vi "PathPlanner_Path_Test.vi"(8 "error in (no error)":errorcluster) -> (0 "error out":errorcluster, 3 "All Passed":bool)   [LabVIEW 2019]
uses:
  <vilib>/Rock Robotics/WPI/ThirdParty/JAS_Junk/TrajLib/Rotation2d_CreateAngle.vi
  <vilib>/Rock Robotics/WPI/ThirdParty/MJansen/PathPlanner/VI/PathPlanner_Waypoint_AutoCtrlPoints.vi
  <vilib>/Rock Robotics/WPI/ThirdParty/JAS_Junk/TrajLib/Pose2d_getTranslation.vi
  <vilib>/Rock Robotics/WPI/ThirdParty/JAS_Junk/TrajLib/Pose2d_getRotation.vi
  <vilib>/Rock Robotics/WPI/ThirdParty/JAS_Junk/TrajLib/Conv_Deg_Radians.vi
  <vilib>/Rock Robotics/WPI/ThirdParty/JAS_Junk/TrajLib/Pose2d_New_TRRO.vi
  <vilib>/Rock Robotics/WPI/ThirdParty/MJansen/PathPlanner/VI/PathPlanner_Path_GetPoint.vi
  <vilib>/Rock Robotics/WPI/ThirdParty/MJansen/PathPlanner/VI/PathPlanner_PathPoint_GetAll.vi
  <vilib>/Rock Robotics/WPI/ThirdParty/MJansen/PathPlanner/VI/PathPlanner_Path_GetIdealStartingState.vi
  <vilib>/Rock Robotics/WPI/ThirdParty/MJansen/PathPlanner/VI/PathPlanner_IdealStartingState_GetAll.vi
  <vilib>/Rock Robotics/WPI/ThirdParty/MJansen/PathPlanner/VI/PathPlanner_Path_IsReversed.vi
  <vilib>/Rock Robotics/WPI/ThirdParty/JAS_Junk/TrajLib/Rotation2d_GetDegrees.vi
  <vilib>/Rock Robotics/WPI/ThirdParty/JAS_Junk/TrajLib/MathUtil_InputModulus.vi
  <vilib>/Rock Robotics/WPI/ThirdParty/MJansen/PathPlanner/VI/PathPlanner_Path_GetInitialHeading.vi
  <vilib>/Rock Robotics/WPI/ThirdParty/JAS_Junk/TrajLib/Translation2d_Minus.vi
  <vilib>/Rock Robotics/WPI/ThirdParty/JAS_Junk/TrajLib/Translation2d_Create_DistAng.vi
  <vilib>/Rock Robotics/WPI/ThirdParty/JAS_Junk/TrajLib/Translation2d_GetDistance.vi
  <vilib>/Rock Robotics/WPI/ThirdParty/MJansen/PathPlanner/VI/PathPlanner_Waypoint_AutoCtrlDistFactor.vi
  <vilib>/Rock Robotics/WPI/ThirdParty/JAS_Junk/TrajLib/Translation2d_Plus.vi
  <vilib>/Rock Robotics/WPI/ThirdParty/JAS_Junk/TrajLib/Rotation2d_GetRadians.vi
  <vilib>/Rock Robotics/WPI/ThirdParty/JAS_Junk/TrajLib/Translation2d_GetAngle.vi
  <vilib>/Rock Robotics/WPI/ThirdParty/JAS_Junk/TrajLib/Rotation2d_GetAngleCosSin.vi
  <vilib>/Rock Robotics/WPI/ThirdParty/JAS_Junk/TrajLib/Util_CalcDist.vi
  <vilib>/Rock Robotics/WPI/ThirdParty/JAS_Junk/TrajLib/Translation2d_GetXY.vi
  <vilib>/Rock Robotics/WPI/ThirdParty/JAS_Junk/TrajLib/Rotation2d_CreateXY.vi
  <vilib>/Rock Robotics/WPI/ThirdParty/JAS_Junk/TrajLib/Trajectory_Library.lvlib
  <vilib>/Rock Robotics/WPI/ThirdParty/MJansen/PathPlanner/PathPlanner24.lvlib
panel:
  out "Error 2":bool
  out "Error":bool
  out "Passed 3":bool
  out "Passed 2":bool
  out "Passed 1":bool
  # "DifferentialStartingPose"
  # "HolomonicStartingPoseSet"
  # "HolomonicStartingPose Null"
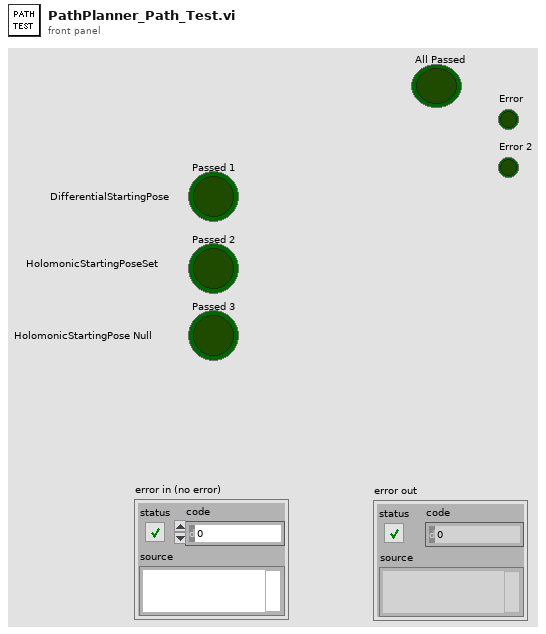
[diagram p1: front panel]
types:
  T1 = typedef "Trajectory_Library.lvlib/TRANSLATION2D.ctl" = cluster{"X":dbl, "Y":dbl}
  T2 = typedef "Trajectory_Library.lvlib/ROTATION2D.ctl" = cluster{"VALUE":dbl, "COS":dbl, "SIN":dbl}
  T3 = typedef "Trajectory_Library.lvlib/POSE2D.ctl" = cluster{"TRANSLATION":T1, "ROTATION":T2}
  T4 = typedef "PathPlanner24.lvlib/PathPlannerPathConstraints.ctl" = cluster{"MaxVelocityMps;":dbl, "MaxAccelerationMpsSq;":dbl, "MaxAngularVelRadPsEc;":dbl, "MaxAngularAccRadPSecSq":dbl, "Exists":bool, "Unlimited":bool, "NominalVoltageVolts":dbl}
  T5 = typedef "PathPlanner24.lvlib/PathPlannerGoalEndState.ctl" = cluster{"VelocityMPS":dbl, "Rotation":T2}
  T6 = typedef "PathPlanner24.lvlib/PathPlannerIdealStartingState.ctl" = cluster{"VelocityMPS":dbl, "Rotation":T2}
  T7 = typedef "PathPlanner24.lvlib/PathPlannerWaypoint.ctl" = cluster{"prevControl":T1, "anchor":T1, "nextControl":T1, "PrevExists":bool, "NextExists":bool}
  T8 = typedef "PathPlanner24.lvlib/PathPlannerPath.ctl" = cluster{"Reversed":bool, "RotationTargets":T9[], "ConstraintZones":T10[], "EventMarkers":T11[], "GlobalConstraints":T4, "GoalEndState":T5, "AllPoints":T14[], "Name":string, "Waypoints":T7[], "PointTowardsZones":T15[], "IdealStartingState":T6, "IsChoreoPath":bool, "PreventFlipping":bool}
  T9 = typedef "PathPlanner24.lvlib/PathPlannerRotationTarget.ctl" = cluster{"position":dbl, "rotation":T2, "Exists":bool}
  T10 = typedef "PathPlanner24.lvlib/PathPlannerConstraintsZone.ctl" = cluster{"minPosition":dbl, "maxPosition":dbl, "Constraints":T4, "Present":bool}
  T11 = typedef "PathPlanner24.lvlib/PathPlannerEventMarker.ctl" = cluster{"Position":dbl, "Command":T12, "TriggerName":string, "EndPosition":dbl}
  T12 = typedef "PathPlanner24.lvlib/PathPlannerCommandUtil.ctl" = cluster{"waitTime":dbl, "name":string, "pathName":string, "commands":cluster{"type":T13, "waitTime":dbl, "name":string, "pathName":string}[], "type":T13}
  T13 = typedef "PathPlanner24.lvlib/PathPlanner_CommandUtilType_ENUM.ctl" = enum16{"Unknown", "Wait", "Named", "Path", "Sequential", "Parallel", "Race", "Deadline"}
  T14 = typedef "PathPlanner24.lvlib/PathPlannerPathPoint.ctl" = cluster{"Position":T1, "DistAlongPath":dbl, "MaxV":dbl, "Constraints":T4, "RotationTarget":T9, "WaypointRelativePos":dbl}
  T15 = typedef "PathPlanner24.lvlib/PathPlannerPointTowardsZone.ctl" = cluster{"RotationOffset":T2, "Name":string, "TargetPosition":T1, "MinPosition":dbl, "MaxPosition":dbl}
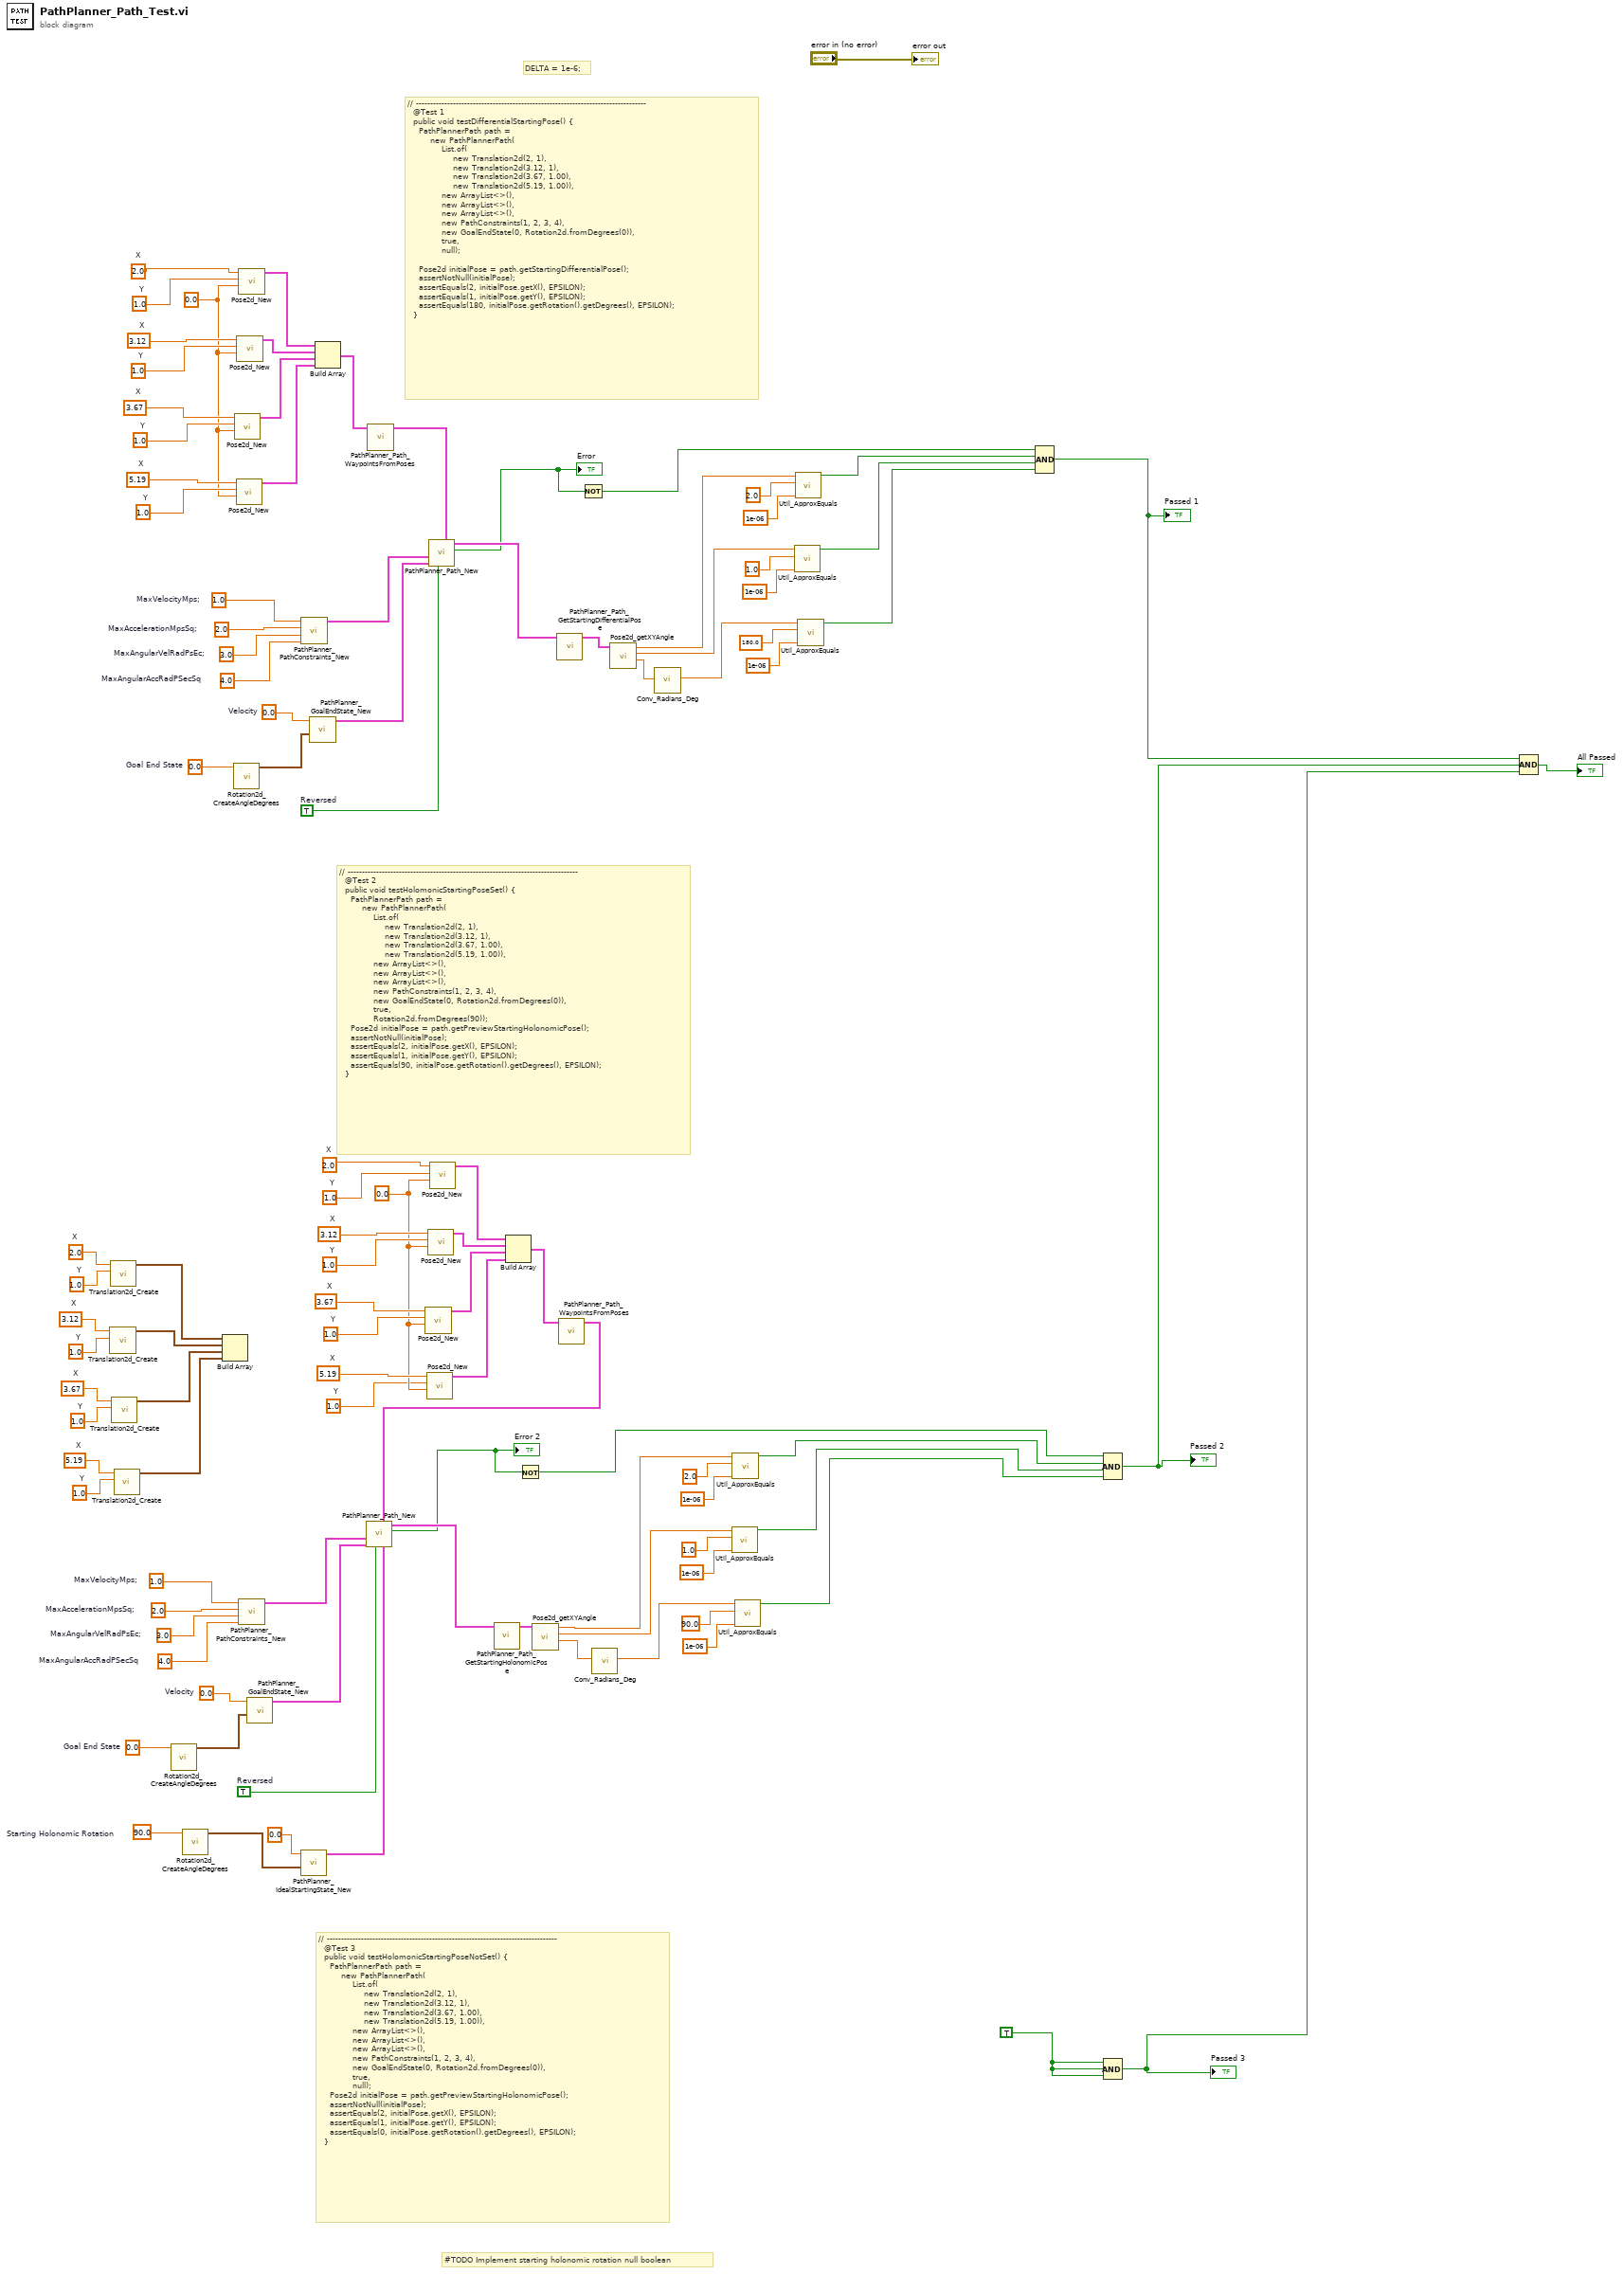
[diagram p0: block diagram]
diagram:
  w12 = 0.0 ("Heading")
  w13 = 5.19  # X
  w6 = 1.0  # Y
  w19 = 2.0  # X
  w18 = 1.0  # Y
  w15 = 3.67  # X
  w14 = 1.0  # Y
  w17 = 3.12  # X
  w16 = 1.0  # Y
  w27 = 0.0 ("Heading")
  w36 = TRUE
  w46 = 90.0  # Starting Holonomic Rotation
  w51 = 0.0  # Velocity
  w53 = 0.0  # Goal End State
  w54 = TRUE  # Reversed
  w60 = 5.19  # X
  w59 = 1.0  # Y
  w62 = 2.0  # X
  w61 = 1.0  # Y
  w64 = 3.67  # X
  w63 = 1.0  # Y
  w66 = 3.12  # X
  w65 = 1.0  # Y
  w72 = 1.0  # MaxVelocityMps;
  w73 = 2.0  # MaxAccelerationMpsSq;
  w74 = 3.0  # MaxAngularVelRadPsEc;
  w75 = 4.0  # MaxAngularAccRadPSecSq
  w87 = 0.0  # Velocity
  w89 = 0.0  # Goal End State
  w90 = TRUE  # Reversed
  w29 = 5.19  # X
  w28 = 1.0  # Y
  w35 = 2.0  # X
  w34 = 1.0  # Y
  w31 = 3.67  # X
  w30 = 1.0  # Y
  w33 = 3.12  # X
  w32 = 1.0  # Y
  w97 = 1.0  # MaxVelocityMps;
  w98 = 2.0  # MaxAccelerationMpsSq;
  w99 = 3.0  # MaxAngularVelRadPsEc;
  w100 = 4.0  # MaxAngularAccRadPSecSq
  # "#TODO Implement starting holonomic rotation null boolean"
  # "// ---------------------------------------------------------------------------------\n  @Test 3\n  public void testHolomonicStartingPoseNotSet() {\n    PathPlannerPath path =\n        new PathPlannerPath(\n            List.of(\n                new Translation2d(2, 1),\n                new Translation2d(3.12, 1),\n                new Translation2d(3.67, 1.00),\n                new Translation2d(5.19, 1.00)),\n            new ArrayList<>(),\n            new ArrayList<>(),\n            new ArrayList<>(),\n            new PathConstraints(1, 2, 3, 4),\n            new GoalEndState(0, Rotation2d.fromDegrees(0)),\n            true,\n            null);\n    Pose2d initialPose = path.getPreviewStartingHolonomicPose();\n    assertNotNull(initialPose);\n    assertEquals(2, initialPose.getX(), EPSILON);\n    assertEquals(1, initialPose.getY(), EPSILON);\n    assertEquals(0, initialPose.getRotation().getDegrees(), EPSILON);\n  }"
  # "// ---------------------------------------------------------------------------------\n  @Test 2\n  public void testHolomonicStartingPoseSet() {\n    PathPlannerPath path =\n        new PathPlannerPath(\n            List.of(\n                new Translation2d(2, 1),\n                new Translation2d(3.12, 1),\n                new Translation2d(3.67, 1.00),\n                new Translation2d(5.19, 1.00)),\n            new ArrayList<>(),\n            new ArrayList<>(),\n            new ArrayList<>(),\n            new PathConstraints(1, 2, 3, 4),\n            new GoalEndState(0, Rotation2d.fromDegrees(0)),\n            true,\n            Rotation2d.fromDegrees(90));\n    Pose2d initialPose = path.getPreviewStartingHolonomicPose();\n    assertNotNull(initialPose);\n    assertEquals(2, initialPose.getX(), EPSILON);\n    assertEquals(1, initialPose.getY(), EPSILON);\n    assertEquals(90, initialPose.getRotation().getDegrees(), EPSILON);\n  }"
  # "// ---------------------------------------------------------------------------------\n  @Test 1\n  public void testDifferentialStartingPose() {\n    PathPlannerPath path =\n        new PathPlannerPath(\n            List.of(\n                new Translation2d(2, 1),\n                new Translation2d(3.12, 1),\n                new Translation2d(3.67, 1.00),\n                new Translation2d(5.19, 1.00)),\n            new ArrayList<>(),\n            new ArrayList<>(),\n            new ArrayList<>(),\n            new PathConstraints(1, 2, 3, 4),\n            new GoalEndState(0, Rotation2d.fromDegrees(0)),\n            true,\n            null);\n\n    Pose2d initialPose = path.getStartingDifferentialPose();\n    assertNotNull(initialPose);\n    assertEquals(2, initialPose.getX(), EPSILON);\n    assertEquals(1, initialPose.getY(), EPSILON);\n    assertEquals(180, initialPose.getRotation().getDegrees(), EPSILON);\n  }"
  # "DELTA = 1e-6;"
  n1 = call <vilib>:"Translation2d_Create.vi"("Y"=w65, "X"=w66) -> ("TRANSLATION"=w57:T1)  [unwired: 9 in]
  n2 = call <vilib>:"Translation2d_Create.vi"("Y"=w61, "X"=w62) -> ("TRANSLATION"=w58:T1)  [unwired: 9 in]
  n3 = call <vilib>:"Translation2d_Create.vi"("Y"=w63, "X"=w64) -> ("TRANSLATION"=w56:T1)  [unwired: 9 in]
  n4 = call <vilib>:"Translation2d_Create.vi"("Y"=w59, "X"=w60) -> ("TRANSLATION"=w55:T1)  [unwired: 9 in]
  n5 = call <vilib>:"Rotation2d_CreateAngleDegrees.vi"("Angle_Degrees"=w53) -> ("ROTATION"=w52:T2)  [unwired: 10 in]
  n6 = call <vilib>:"Rotation2d_CreateAngleDegrees.vi"("Angle_Degrees"=w46) -> ("ROTATION"=w1:T2)  [unwired: 10 in]
  n7 = Build Array(w58, w57, w56, w55) -> ()  [unwired: 1 out]
  n8 = call <vilib>:"Rotation2d_CreateAngleDegrees.vi"("Angle_Degrees"=w89) -> ("ROTATION"=w88:T2)  [unwired: 10 in]
  n9 = call <vilib>:"Pose2d_New.vi"("Heading"=w27, "Y"=w30, "X"=w31) -> ("out POSe"=w24:T3)  [unwired: 8 in]
  n10 = call <vilib>:"Pose2d_New.vi"("Heading"=w27, "Y"=w28, "X"=w29) -> ("out POSe"=w23:T3)  [unwired: 8 in]
  n11 = call <vilib>:"Pose2d_New.vi"("Heading"=w27, "Y"=w32, "X"=w33) -> ("out POSe"=w25:T3)  [unwired: 8 in]
  n12 = call <vilib>:"Pose2d_New.vi"("Heading"=w27, "Y"=w34, "X"=w35) -> ("out POSe"=w26:T3)  [unwired: 8 in]
  n13 = call <vilib>:"PathPlanner_PathConstraints_New.vi"("MaxAngularAccRadPSecSq"=w75, "MaxAngularVelRadPsEc;"=w74, "MaxAccelerationMpsSq;"=w73, "MaxVelocityMps;"=w72) -> ("PathPlannerConstraints"=w67:T4)  [unwired: 7 in]
  n14 = call <vilib>:"PathPlanner_GoalEndState_New.vi"("Rotation"=w52, "VelocityMPS"=w51) -> ("GoalEndState"=w50:T5)  [unwired: 9 in]
  n15 = call <vilib>:"PathPlanner_IdealStartingState_New.vi"("Rotation"=w1, "VelocityMPS"=0.0) -> ("IdealStartingState"=w3:T6)  [unwired: 9 in]
  n16 = call <vilib>:"PathPlanner_PathConstraints_New.vi"("MaxAngularAccRadPSecSq"=w100, "MaxAngularVelRadPsEc;"=w99, "MaxAccelerationMpsSq;"=w98, "MaxVelocityMps;"=w97) -> ("PathPlannerConstraints"=w91:T4)  [unwired: 7 in]
  n17 = call <vilib>:"PathPlanner_GoalEndState_New.vi"("Rotation"=w88, "VelocityMPS"=w87) -> ("GoalEndState"=w86:T5)  [unwired: 9 in]
  n18 = Build Array(w26, w25, w24, w23) -> (w22:T3[])
  n19 = call <vilib>:"PathPlanner_Path_WaypointsFromPoses.vi"("Poses"=w22) -> ("Waypoints"=w21:T7[])  [unwired: 9 in, 1 out]
  n20 = call <vilib>:"Pose2d_New.vi"("Heading"=w12, "Y"=w14, "X"=w15) -> ("out POSe"=w9:T3)  [unwired: 8 in]
  n21 = call <vilib>:"Pose2d_New.vi"("Heading"=w12, "Y"=w6, "X"=w13) -> ("out POSe"=w8:T3)  [unwired: 8 in]
  n22 = call <vilib>:"Pose2d_New.vi"("Heading"=w12, "Y"=w16, "X"=w17) -> ("out POSe"=w10:T3)  [unwired: 8 in]
  n23 = call <vilib>:"PathPlanner_Path_New.vi"("Waypoints"=w21, "Reversed"=w90, "GoalEndState"=w86, "GlobalConstraints"=w91) -> ("Error"=w20:bool, "PathPlannerPath"=w84:T8)  [unwired: 6 in]
  "Error" <- w20
  n24 = call <vilib>:"Pose2d_New.vi"("Heading"=w12, "Y"=w18, "X"=w19) -> ("out POSe"=w11:T3)  [unwired: 8 in]
  n25 = Build Array(w11, w10, w9, w8) -> (w7:T3[])
  n26 = call <vilib>:"PathPlanner_Path_GetStartingDifferentialPose.vi"("PathPlannerPath"=w84) -> ("StartingDifferentialPose"=w83:T3)  [unwired: 10 in]
  n27 = call <vilib>:"PathPlanner_Path_WaypointsFromPoses.vi"("Poses"=w7) -> ("Waypoints"=w5:T7[])  [unwired: 9 in, 1 out]
  n28 = call <vilib>:"PathPlanner_Path_New.vi"("IdealStartingState"=w3, "Waypoints"=w5, "Reversed"=w54, "GoalEndState"=w50, "GlobalConstraints"=w67) -> ("Error"=w4:bool, "PathPlannerPath"=w45:T8)  [unwired: 5 in]
  "Error 2" <- w4
  n29 = call <vilib>:"PathPlanner_Path_GetStartingHolonomicPose.vi"("PathPlannerPath"=w45) -> ("StartingHolonomicPose"=w44:T3)  [unwired: 10 in]
  n30 = Not(x=w4) -> (.not. x?=w40:bool)
  n31 = call <vilib>:"Pose2d_getXYAngle.vi"("in POSE"=w44) -> ("Angle"=w41:dbl, "Y"=w42:dbl, "X"=w43:dbl)  [unwired: 8 in]
  n32 = Not(x=w20) -> (.not. x?=w85:bool)
  n33 = call <vilib>:"Conv_Radians_Deg.vi"("Radians"=w41) -> ("Degrees"=w47:dbl)  [unwired: 10 in]
  n34 = call <vilib>:"Pose2d_getXYAngle.vi"("in POSE"=w83) -> ("Angle"=w82:dbl, "Y"=w80:dbl, "X"=w81:dbl)  [unwired: 8 in]
  n35 = call <vilib>:"Conv_Radians_Deg.vi"("Radians"=w82) -> ("Degrees"=w77:dbl)  [unwired: 10 in]
  n36 = call <vilib>:"Util_ApproxEquals.vi"("Tolerance"=1e-06, "Value 2"=1.0, "Value 1"=w42) -> ("ApproxEquals"=w38:bool)  [unwired: 8 in]
  n37 = call <vilib>:"Util_ApproxEquals.vi"("Tolerance"=1e-06, "Value 2"=2.0, "Value 1"=w43) -> ("ApproxEquals"=w39:bool)  [unwired: 8 in]
  n38 = call <vilib>:"Util_ApproxEquals.vi"("Tolerance"=1e-06, "Value 2"=90.0, "Value 1"=w47) -> ("ApproxEquals"=w37:bool)  [unwired: 8 in]
  n39 = call <vilib>:"Util_ApproxEquals.vi"("Tolerance"=1e-06, "Value 2"=1.0, "Value 1"=w80) -> ("ApproxEquals"=w92:bool)  [unwired: 8 in]
  n40 = call <vilib>:"Util_ApproxEquals.vi"("Tolerance"=1e-06, "Value 2"=2.0, "Value 1"=w81) -> ("ApproxEquals"=w104:bool)  [unwired: 8 in]
  n41 = call <vilib>:"Util_ApproxEquals.vi"("Tolerance"=1e-06, "Value 2"=180.0, "Value 1"=w77) -> ("ApproxEquals"=w76:bool)  [unwired: 8 in]
  n42 = Compound Arithmetic op=AND(w85, w104, w92, w76) -> (w103:bool)
  "Passed 1" <- w103
  n43 = Compound Arithmetic op=AND(w40, w39, w38, w37) -> (w102:bool)
  "Passed 2" <- w102
  n44 = Compound Arithmetic op=AND(w36, w36, w36) -> (w101:bool)
  "Passed 3" <- w101
  n45 = Compound Arithmetic op=AND(w103, w102, w101) -> (→"All Passed":bool)
  "error out" <- "error in (no error)"
